vi "FT10xx系列_T2-T3_sample_1.0.3.vi"() -> ()   [LabVIEW 2017]
uses:
  National Instruments/LabVIEW 2017/user.lib/smncsftmt/smncsftmt.lvlib
panel:
  in  "数量":u32
  in  "时间（s）":sgl=1.0
  in  "模式选择":enum32{"单选选项1", "单选选项2"}(radio)
  out "error out":errorcluster
  in  "退出采集 2":bool
  in  "保存文件夹":path=path "D:/siminics"
  out "已连接？":bool
  in  "单选按钮":enum32{"时间停止", "事件停止"}(radio)
  # "FT10XX系列时间标签模式"
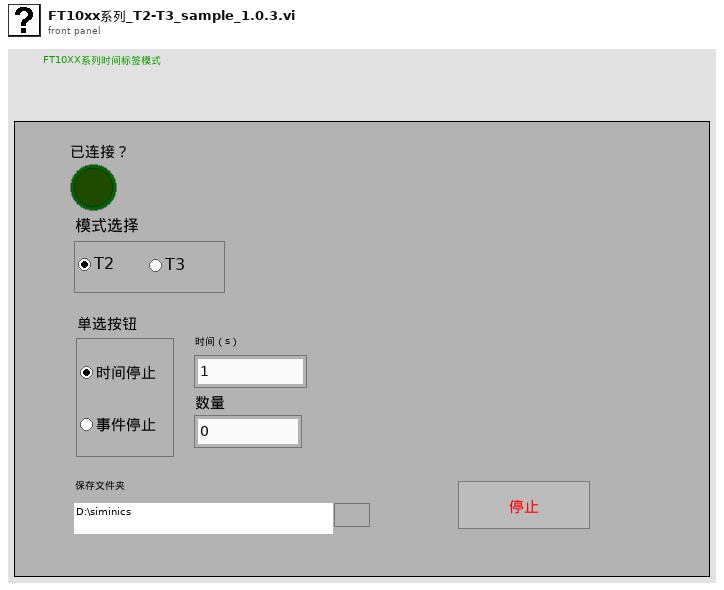
[diagram p1: front panel]
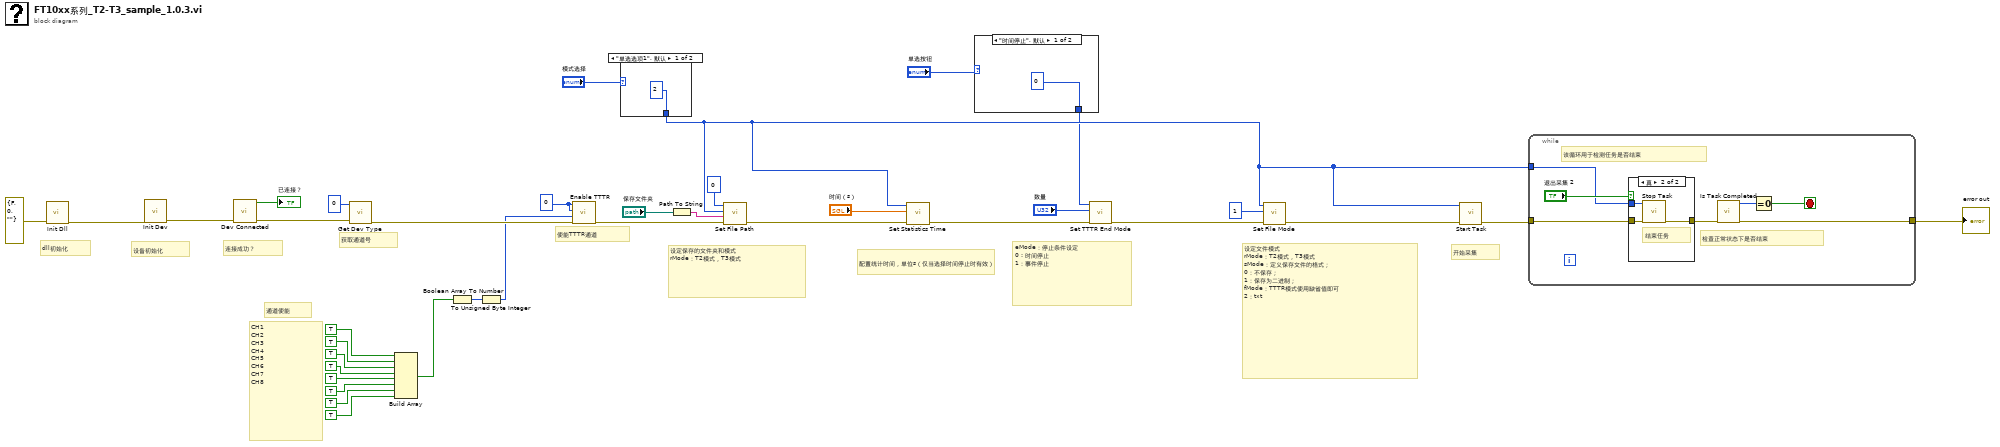
[diagram p0: block diagram]
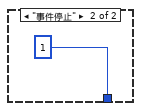
[diagram p2: hidden frame]
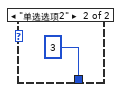
[diagram p3: hidden frame]
diagram:
  w23 = 0 ("brd")
  # "通道使能"
  # "CH1\nCH2\nCH3\nCH4\nCH5\nCH6\nCH7\nCH8"
  # "连接成功？"
  # "设备初始化"
  # "dll初始化"
  # "获取通道号"
  # "开始采集"
  # "设定文件模式\nrMode：T2模式，T3模式\nsMode：定义保存文件的格式；\n0：不保存；\n1：保存为二进制；\nfMode：TTTR模式使用缺省值即可\n2：txt"
  # "eMode：停止条件设定\n0 : 时间停止\n1：事件停止"
  # "配置统计时间，单位s（仅当选择时间停止时有效）"
  # "设定保存的文件夹和模式\nrMode：T2模式，T3模式"
  # "使能TTTR通道"
  n1 = call "Init Dll.vi"("error in (no error)"=errorcluster {"status"=FALSE, "code"=0, "source"=""}) -> ("error out"=w16:errorcluster)  [unwired: 9 in, 1 out]
  n2 = call "Init Dev.vi"("error in (no error)"=w16) -> ("error out"=w15:errorcluster)  [unwired: 9 in, 1 out]
  n3 = call "Dev Connected.vi"("error in (no error)"=w15) -> ("error out"=w13:errorcluster, "function return"=→"已连接？":bool)  [unwired: 9 in]
  n4 = call "Get Dev Type.vi"("error in (no error)"=w13, "nDevId"=0) -> ("error out"=w25:errorcluster)  [unwired: 7 in, 2 out]
  n5 = Build Array(TRUE, TRUE, TRUE, TRUE, TRUE, TRUE, TRUE, TRUE) -> (w2:bool[])
  n6 = Boolean Array To Number(Boolean array=w2) -> (number=w11:u32)
  n7 = To Unsigned Byte Integer(number=w11) -> (unsigned 8bit integer=w1:u8)
  n8 = call "Enable TTTR.vi"("error in (no error)"=w25, "uMask16"=w1, "nBoard"=w23, "nDevId"=w23) -> ("error out"=w34:errorcluster)  [unwired: 6 in, 1 out]
  n9 = case shown="\"单选选项1\", 默认" "模式选择" {
    tunnel: [u16 2 u16 3] -> w21
    frame "单选选项1", Default {
    }
    frame "单选选项2" {
    }
  }
  n10 = Path To String(path="保存文件夹") -> (string=w36:string)
  n11 = call "Set File Path.vi"("error in (no error)"=w34, "strFilePath"=w36, "nRunMode"=w21, "nDevId"=0) -> ("error out"=w33:errorcluster)  [unwired: 6 in, 1 out]
  n12 = call "Set Statistics Time.vi"("error in (no error)"=w33, "Times"="时间（s）", "nRunMode"=w21) -> ("error out"=w31:errorcluster)  [unwired: 7 in, 1 out]
  n13 = case shown="\"时间停止\", 默认" "单选按钮" {
    tunnel: [0 1] -> w18
    frame "时间停止", Default {
    }
    frame "事件停止" {
    }
  }
  n14 = call "Set TTTR End Mode.vi"("error in (no error)"=w31, "uEvents64"="数量", "nEndMode"=w18) -> ("error out"=w30:errorcluster)  [unwired: 7 in, 1 out]
  n15 = call "Set File Mode.vi"("error in (no error)"=w30, "nSaveMode"=1 ("rMode"), "nRunMode"=w21) -> ("error out"=w28:errorcluster)  [unwired: 7 in, 1 out]
  n16 = call "Start Task.vi"("error in (no error)"=w28, "nRunMode"=w21) -> ("error out"=w27:errorcluster)  [unwired: 8 in, 1 out]
  n17 = while {
    tunnel: w27 -> [w47]
    tunnel: [w43] -> w26
    tunnel: w21 -> [w44]
    stop <- w41 stop-if-true
    # "检查正常状态下是否结束"
    # "该循环用于检测任务是否结束"
    n18 = case shown="真" "退出采集 2" {
      tunnel: [w48 w50] -> w46
      tunnel: w47 -> [w48 w51]
      tunnel: w44 -> [_ w49]
      frame False {
      }
      frame True {
        # "结束任务"
        n19 = call "Stop Task.vi"("error in (no error)"=w51, "nRunMode"=w49) -> ("error out"=w50:errorcluster)  [unwired: 8 in, 1 out]
      }
    }
    n20 = call "Is Task Completed.vi"("error in (no error)"=w46) -> ("error out"=w43:errorcluster, "function return"=w42:i32)  [unwired: 9 in]
    n21 = Equal To 0?(x=w42) -> (x = 0?=w41:bool)
  }
  "error out" <- w26
